vi "RemoteVI Complex View A.vi"() -> ()   [LabVIEW 2020]
doc: "View A of RemoteVI Complex Fixture.vi, shown in its subpanel Viewer. A small panel of its own: A Text (string), A Gain (numeric), A Apply (latched button). It obtains the named queue RemoteVI Complex Fixture (the fixture writes the vlayout lines of the VI shown in the subpanel). An event loop enqueues one log line per event: value changes of A Text, A Gain and A Apply, key down on A Text, mouse down on all three. A parallel loop waits on the named notifier RemoteVI Complex Fixture and, when it fires or is destroyed, sets the hidden switch A Quit with Value (Signaling), which ends the event loop. The fixture writes the queued lines to its log."
panel:
  in  "A Quit":bool
  in  "A Gain":dbl
  in  "A Text":string
  in  "A Apply":bool
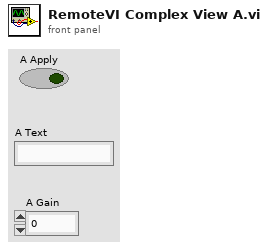
[diagram p1: front panel]
types:
  T1 = typedef "eventvkey.ctl" = enum16{"ASCII", "Enter", "Return", "Shift", "Ctrl", "Alt", "Cmd", "Opt", "Caps", "NumLock", "Clear", "Break", "Up", "Down", "Left", "Right", "Insert", "Delete", "Home", "End", "PageUp", "PageDown", "Escape", "Help", "Pause", "ScrollLock", "F1", "F2", "F3", "F4", "F5", "F6", "F7", "F8", "F9", "F10", "F11", "F12", "F13", "F14", "F15", "F16", "F17", "F18", "F19", "F20", "F21", "F22", "F23", "F24", "Play", "VolumeUp", "VolumeDown", "Mute", "Two Byte Char"}
  T2 = cluster{"Shift":bool, "Ctrl":bool, "Alt":bool, "Cmd":bool, "Opt":bool}
  T3 = typedef "LVPoint32TypeDef.ctl" = cluster{"Horizontal":i32, "Vertical":i32}
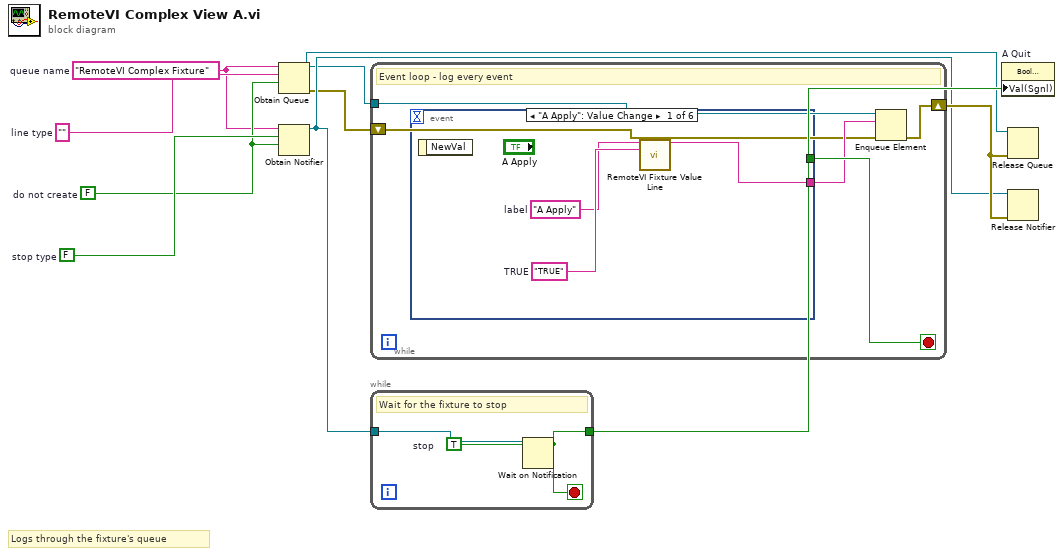
[diagram p0: block diagram]
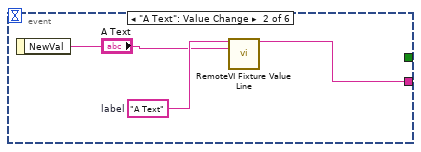
[diagram p2: hidden frame]
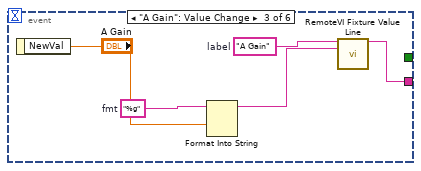
[diagram p3: hidden frame]
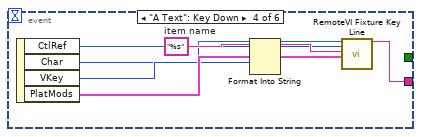
[diagram p4: hidden frame]
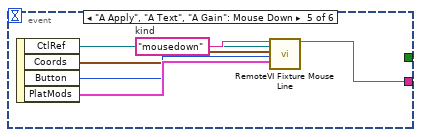
[diagram p5: hidden frame]
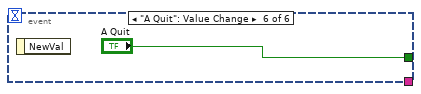
[diagram p6: hidden frame]
diagram:
  w6 = FALSE  # stop type
  w3 = FALSE  # do not create
  w2 = ""  # line type
  w1 = "RemoteVI Complex Fixture"  # queue name
  # "Logs through the fixture's queue"
  n1 = Obtain Queue(name (unnamed)=w1, element data type=w2, create if not found? (T)=w3) -> (queue out=w4:refnum<queue>, error out=w5:errorcluster)  [unwired: 2 in, 1 out]
  n2 = Obtain Notifier(name (unnamed)=w1, notification data type=w6, create if not found? (T)=w3) -> (notifier out=w7:refnum<notifier>)  [unwired: 1 in, 2 out]
  n3 = while {
    tunnel: w4 -> [w10]
    shift-right: [w12] -> w8
    shift-left: w5 -> [w11]
    stop <- w14 stop-if-true
    # "Event loop - log every event"
    n4 = event shown="[0] \"A Apply\": Value Change" {
      selector: _ -> [_ _ _ _ _ _]
      dyn-events: _ -> [_ _ _ _ _ _]
      timeout: _ -> [_ _ _ _ _ _]
      tunnel: [_ _ _ _ _ "A Quit"] -> w14
      tunnel: [w17 w20 w25 w32 w38 _] -> w13
      event "A Apply": Value Change {
        w16 = "TRUE"  # TRUE
        w15 = "A Apply"  # label
        n5 = event-data() -> ()  [unwired: 1 in, 1 out]
        n6 = call "RemoteVI Fixture Value Line.vi"("label"=w15, "value"=w16) -> ("line"=w17:string)  [unwired: 12 in, 1 out]
      }
      event "A Text": Value Change {
        w19 = "A Text"  # label
        n7 = event-data() -> ("NewVal"=w18:string)  [unwired: 1 in]
        n8 = call "RemoteVI Fixture Value Line.vi"("label"=w19, "value"=w18) -> ("line"=w20:string)  [unwired: 12 in, 1 out]
      }
      event "A Gain": Value Change {
        w24 = "A Gain"  # label
        w22 = "%g"  # fmt
        n9 = event-data() -> ("NewVal"=w21:dbl)  [unwired: 1 in]
        n10 = Format Into String(format string=w22, w21) -> (resulting string=w23:string)  [unwired: 2 in, 1 out]
        n11 = call "RemoteVI Fixture Value Line.vi"("label"=w24, "value"=w23) -> ("line"=w25:string)  [unwired: 12 in, 1 out]
      }
      event "A Text": Key Down {
        w30 = "%s"  # item name
        n12 = event-data() -> ("CtlRef"=w26:refnum<vi>, "Char"=w27:i16, "VKey"=w28:T1, "PlatMods"=w29:T2)  [unwired: 1 in]
        n13 = Format Into String(format string=w30, w28) -> (resulting string=w31:string)  [unwired: 2 in, 1 out]
        n14 = call "RemoteVI Fixture Key Line.vi"("CtlRef"=w26, "Char"=w27, "VKey"=w31, "PlatMods"=w29) -> ("line"=w32:string)  [unwired: 14 in, 1 out]
      }
      event "A Apply", "A Text", "A Gain": Mouse Down {
        w37 = "mousedown"  # kind
        n15 = event-data() -> ("CtlRef"=w33:refnum<vi>, "Coords"=w34:T3, "Button"=w35:u16, "PlatMods"=w36:T2)  [unwired: 1 in]
        n16 = call "RemoteVI Fixture Mouse Line.vi"("kind"=w37, "CtlRef"=w33, "Coords"=w34, "Button"=w35, "PlatMods"=w36) -> ("line"=w38:string)  [unwired: 13 in, 1 out]
      }
      event "A Quit": Value Change {
        n17 = event-data() -> ()  [unwired: 1 in, 1 out]
      }
    }
    n18 = Enqueue Element(queue=w10, element=w13, error in (no error)=w11) -> (error out=w12:errorcluster)  [unwired: 1 in, 2 out]
  }
  n19 = while {
    tunnel: [w41] -> w9
    tunnel: w7 -> [w40]
    stop <- w41 stop-if-true
    w41 = TRUE  # stop
    # "Wait for the fixture to stop"
    n20 = Wait on Notification(notifier=w40) -> ()  [unwired: 3 in, 4 out]
  }
  n21 = property on="A Quit" class="Bool (strict)"("Val(Sgnl)"=w9) -> ()  [unwired: 2 in, 2 out]
  n22 = Release Queue(queue=w4, error in (no error)=w8) -> ()  [unwired: 1 in, 3 out]
  n23 = Release Notifier(notifier=w7, error in (no error)=w8) -> ()  [unwired: 1 in, 3 out]
